vi "Define_Last_Point_in_Subtrack-1.vi"(4 "[IN] Statuses":i16[](array[numeric])) -> (1 "[OUT] Index of Problem Point\nin Subtrack (Original)":i32)   [LabVIEW 2017]
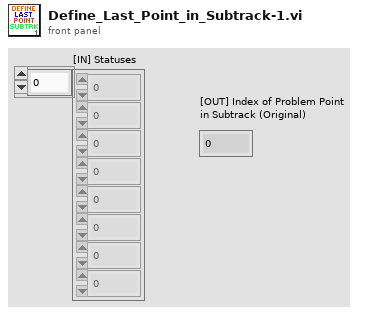
[diagram p1: front panel]
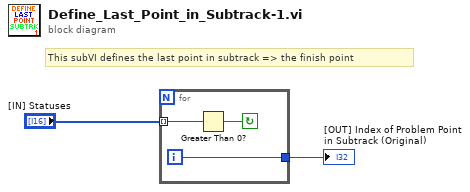
[diagram p0: block diagram]
diagram:
  # "This subVI defines the last point in subtrack => the finish point"
  n1 = for {
    tunnel: "[IN] Statuses" -> [w5] mode=indexing
    tunnel: [w3] -> w1
    i -> [w3]
    stop <- w4 continue-if-true
    n2 = Greater Than 0?(x=w5) -> (x > 0?=w4:bool)
  }
  "[OUT] Index of Problem Point\nin Subtrack (Original)" <- w1
